vi "VM - Arbitrary Data.vi"(6 "var type":u32=128, 7 "VC Handle":T3=-1, 8 "error in":errorcluster, 9 "cmd":T2(ring)=enum."get value", 10 "flattened value":string, 11 "name_spec":string) -> (0 "error out":errorcluster, 1 "err code":T1 items=["No error", "Invalid variable type", "Variable not found", "Variable already exists", "Invalid context handle", "Input error", "Invalid data format", "No history attached", "History already attached", "Invalid history parameters", "Wrong variable name", "Wrong alias name", "Non-unique alias", "Alias not found", "No alias associated", "Alias already associated", "Wrong context name", "Non-unique context name", "Context name not found", "Invalid parameter", "Generic error", "Memory Full", "Unrecognized LV error", "Unknown error code"], 2 "flattened value out":string, 3 "dup name_spec":string, 4 "var type out":u32, 5 "dup VC Handle":T3=-1)   [LabVIEW 2021]
doc: "This VI manages variables that may have an arbitrary data type; both predefined and user-defined data types are supported. Variable values are represented in the Flattened-To-String format, except for String variables, which use the native LabVIEW string representation. You can use this VI as a basis to build VIs that manage variables of custom data types. Refer to the VI help for more details.\n\n<b>VC Handle</b> specifies the handle of the variable context. This input is ignored if the <b>name_spec</b> control refers to a variable by an alias during 'get value', 'set value', and 'destroy' actions.\n\n<b>name_spec</b> is the name specifier of the desired variable. Usually, it is merely a variable name; however, its generic format is '[name][=alias]', where either 'name' or '=alias' can be omitted but not both.\n\n<b>cmd</b> control specifies the action to be performed on the variable. Possible actions are 'create', 'destroy', 'get value', and 'set value'.\n\n<b>flattened value</b> control specifies the value to be written to the variable; it is only used during 'set value' or 'create' actions. <b>flattened value out</b> indicator returns the value that has been read from the variable. Values of all data types are presented in the Flattened-To-String format with the exception of the String type. For the predefined data types, the VI checks the consistency of the data type code and value format, and returns an error in case of a mismatch.\n\n<b>var type</b> is a required control that specifies the data type code of the desired variable. VarMan strictly uses a data type code. However, you can pass -1 to this input to read a variable value of an arbitrary data type, in which case the <b>var type out</b> indicator will return the actual data type code. Passing a data type code of -1 during the 'set value' or 'create' actions will cause the VI to return an error.\n\n<b>err code</b> indicator returns a VarMan Engine error code.\n\n::: CalcExpress Toolkit :::\nCopyright (c) 2000-2026 Konstantin Shifershteyn. All rights reserved."
uses:
  cetypes.llb/VarMan Variable Context Handle.ctl
  cetypes.llb/VarMan Error Code.ctl
  cersrc/celveng32.dll
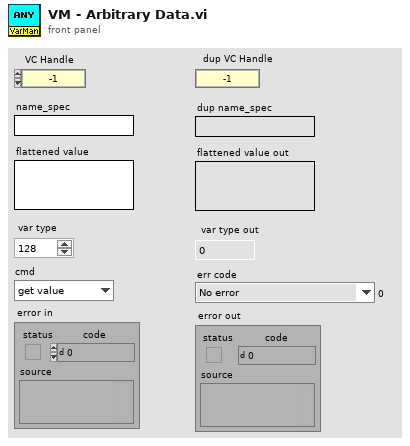
[diagram p1: front panel]
types:
  T1 = typedef "VarMan Error Code.ctl" = u16
  T2 = enum16{"create", "destroy", "set value", "get value"}
  T3 = typedef "VarMan Variable Context Handle.ctl" = i32
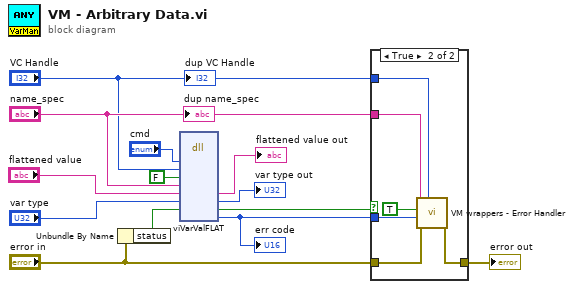
[diagram p0: block diagram]
diagram:
  n1 = Unbundle By Name("error in") -> ("status"=w8:bool)
  n2 = dll-call lib="C:/LV Projects/CalcExpress 40 LV2021/vi.lib/addons/CalcExpress/cersrc/celveng*.dll" fn="viVarValFLAT"("cmd"="cmd", "vch"="VC Handle", "gbl"=FALSE ("global? (F)"), "name"="name_spec", "val"="flattened value", "type"="var type", "errf"=w8) -> ("val"=→"flattened value out":string, "type"=→"var type out":u32, "errf"=w1:bool, "err code"=w3:T1)  [unwired: 9 in, 2 out]
  "err code" <- w3
  n3 = case shown="True" w1 {
    tunnel: [w14 w20] -> w13
    tunnel: "error in" -> [w14 w19]
    tunnel: w3 -> [_ w18]
    tunnel: "name_spec" -> [_ w16]
    tunnel: "VC Handle" -> [_ w15]
    frame False {
    }
    frame True {
      n4 = call "VM wrappers - Error Handler.vi"("VC Handle"=w15, "error before"=w19, "VarMan error"=w18, "show name spec (F)"=TRUE, "name spec"=w16) -> ("error out"=w20:errorcluster)  [unwired: 5 in, 1 out]
    }
  }
  "error out" <- w13
  "dup VC Handle" <- "VC Handle"
  "dup name_spec" <- "name_spec"
